vi "PicoScope5000aExampleStreamingMSO.vi"() -> ()   [LabVIEW 2016]
doc: "This example demonstrates how to use the PicoScope Labview library to stream data from a PicoScope 5000 Series Device"
uses:
  ps5000a.dll
  <vilib>/Waveform/DWDTOps.llb/DWDT Analog to Digital.vi
panel:
  out "Analog Channels":T1(graph)
  out "Raw Sample Interval (sec)":dbl=1.0000000130088963e-06 format="%#.5p"
  out "Max ADC value":i16
  out "Chunk time":u32
  out "Elapsed time":dbl
  in  "Poll time (ms)":u32=10 min=1 max=1000 step=1
  in  "Data file":path=path "PicoScope5000aExampleStreaming ChA Data"
  out "size(s)":i32
  out "Queue depth":i32(graph)
  out "queue depth":i32
  in  "Buffer and Transfer Settings":T2={"startIndex"=0, "Samples"=1000000, "Down Sample Ratio"=1, "Down-Sample Mode"=0} {"Down-Sample Mode" items=["None"=0, "Aggregate"=1, "Decimate"=2, "Average"=4]; "Down Sample Ratio" step=1; "Samples" format="%_6p"}
  in  "Channel A Settings":T3={"Enabled"=TRUE, "Coupling"=1, "Range"=6, "Analogue Offset"=0.0, "Bandwidth Limit"=0} {"Bandwidth Limit" items=["Full", "20MHz"]; "Range" items=["10 mV", "20 mV", "50 mV", "100 mV", "200 mV", "500 mV", "1 V", "2 V", "5 V", "10 V", "20 V"]; "Coupling" items=["AC", "DC"]}
  out "USB Powered":bool=TRUE
  out "USB 3.0 device on non-USB 3.0 Port":bool=TRUE
  out "TriggeredAt (In Buffer)":u32 format="%#.6p"
  out "TriggeredAt (Total samples)":u32 format="%#.6p"
  in  "Acquisition Settings":T4={"Auto Stop"=TRUE, "Desired Sample Interval"=1, "Pre-trigger Samples"=0, "Post-trigger Samples"=1000000, "Down-Sample Ratio"=1, "Down-Sample Mode"=0, "Time Units"=3} {"Time Units" items=["Nanoseconds (ns)"=2, "Microseconds (us)"=3, "Milliseconds (ms)"=4, "Seconds (s)"=5]; "Down-Sample Mode" items=["None"=0, "Aggregate"=1, "Decimate"=2, "Average"=4]; "Post-trigger Samples" format="%#.6p"; "Pre-trigger Samples" format="%#_6p"}
  out "Port 0":digitalwaveform(graph)={"t0"=timestamp(0 s since 1904-01-01), "dt"=1.0000000130088963e-06, "Y"={"transitions"=[], "data"=[]}}
  in  "Port 0 Settings":cluster{"Enabled":bool, "Logic Level":i16}={"Enabled"=FALSE, "Logic Level"=9830} {"Logic Level" items=["1.5V TTL"=9830, "2.5V CMOS"=16383]}
  in  "Trigger Settings":T5={"Trigger Enabled"=FALSE, "Trigger Source"=enum."Channel A", "Trigger Threshold (volts)"=0.0, "Trigger Direction"=2, "Trigger Delay (samples)"=0, "Auto Trigger Time (ms)"=1000} {"Trigger Direction" items=["Rising"=2, "Falling"=3]}
  out "Triggered":bool
  out "DownSample Interval (sec)":dbl=1.0000000130088963e-06 format="%#.5p"
  out "Total Samples":u32 format="%#.6p"
  out "Auto Stopped":bool
  in  "Serial Number":string
  in  "Open Using Serial Number":bool
  out "Number of Samples per Capture":u32 format="%#.6p"
  in  "Resolution":i32(ring) items=["8-bit", "12-bit", "14-bit", "15-bit (max. 2 ch.)", "16-bit (max. 1 ch.)"]
  in  "Apply  Settings":bool
  in  "stop":bool
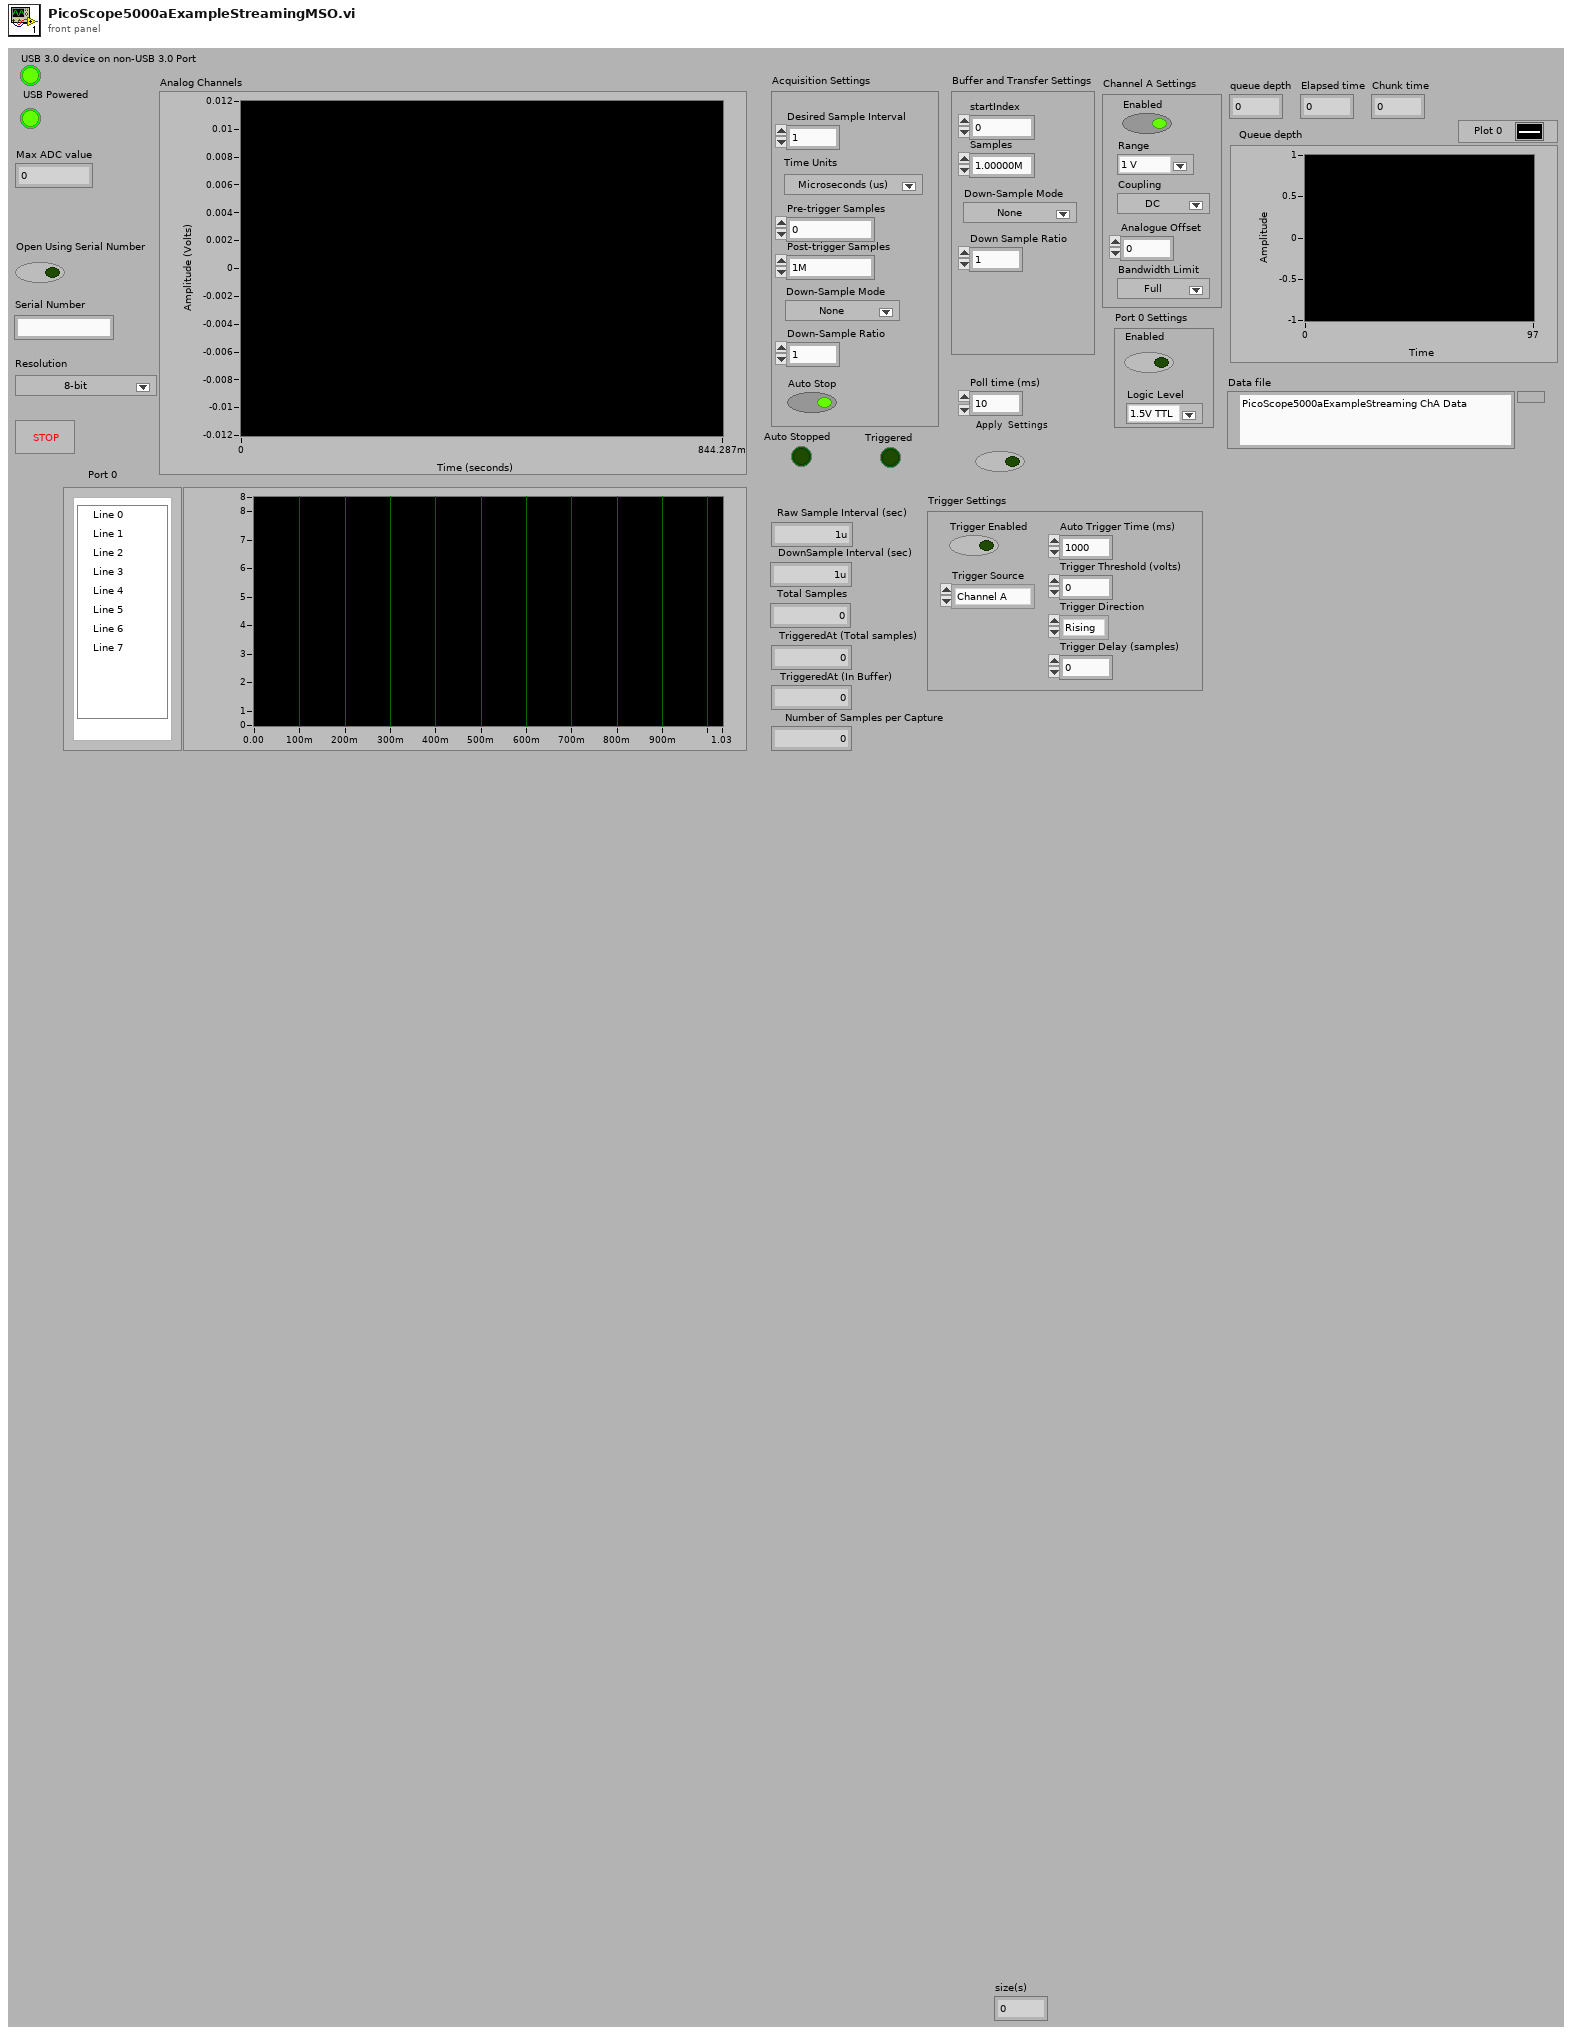
[diagram p1: front panel]
types:
  T1 = cluster{i32, "DownSample Interval (sec)":dbl, "Data":dbl[]}
  T2 = cluster{"startIndex":u64, "Samples":u64, "Down Sample Ratio":u64, "Down-Sample Mode":u32}
  T3 = cluster{"Enabled":bool, "Coupling":i16, "Range":u16, "Analogue Offset":sgl, "Bandwidth Limit":u32}
  T4 = cluster{"Auto Stop":bool, "Desired Sample Interval":u32, "Pre-trigger Samples":u32, "Post-trigger Samples":u32, "Down-Sample Ratio":u32, "Down-Sample Mode":i32, "Time Units":u32}
  T5 = cluster{"Trigger Enabled":bool, "Trigger Source":enum16{"Channel A", "Channel B", "Channel C", "Channel D", "Ext."}, "Trigger Threshold (volts)":dbl, "Trigger Direction":u16, "Trigger Delay (samples)":u32, "Auto Trigger Time (ms)":i16}
  T6 = enum16{"open", "open or create", "create or replace", "create", "open (read-only)"}
  T7 = cluster{"Driver Version":string, "USB Version":string, "Hardware":string, "Variant":string, "Batch and Serial":string, "Cal Date":string, "Kernel Version":string, "Digital HW Version":string, "Analogue HW Version":string, "MSO":bool, "Number of channels":i16}
  T8 = cluster{"Channel A Buffer":i16[], "Channel B Buffer":i16[], "Channel C Buffer":i16[], "Channel D Buffer":i16[], "Channel E Buffer":i16[], "Channel F Buffer":i16[], "Channel G Buffer":i16[], "Channel H Buffer":i16[], "Port 0":i16[], "Port 1":i16[]}
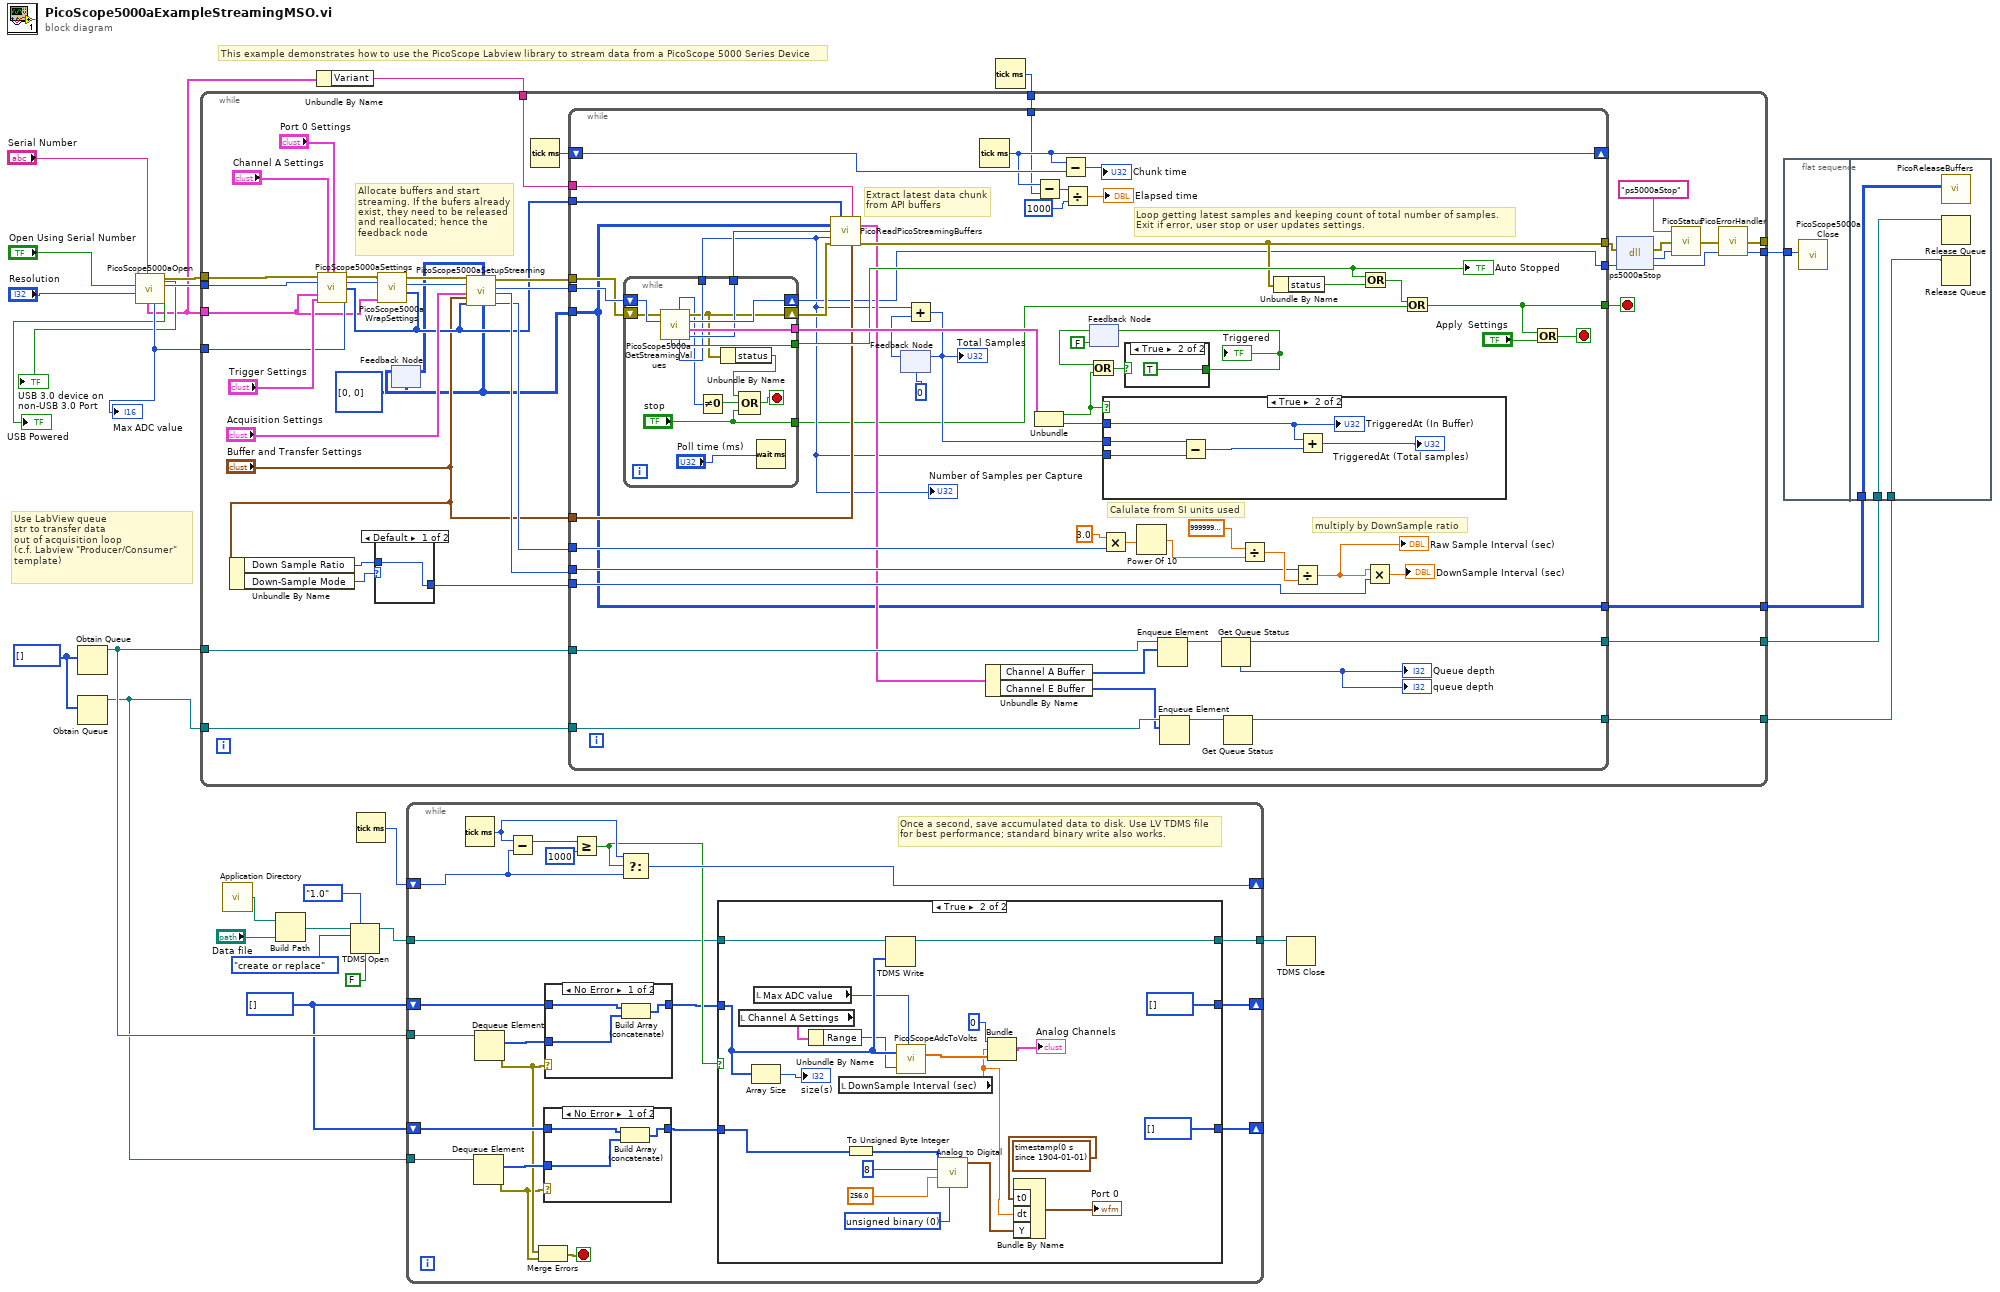
[diagram p0: block diagram]
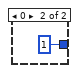
[diagram p5: hidden frame]
diagram:
  w6 = i16[] [] ("History Data")
  w9 = i16[] [] ("History Data")
  # "Use LabView queue\nstr to transfer data\nout of acquisition loop\n(c.f. Labview \"Producer/Consumer\"\ntemplate)"
  # "This example demonstrates how to use the PicoScope Labview library to stream data from a PicoScope 5000 Series Device"
  n1 = Obtain Queue(element data type=w9) -> (queue out=w22:refnum<queue>)  [unwired: 4 in, 2 out]
  n2 = Obtain Queue(element data type=w9) -> (queue out=w7:refnum<queue>)  [unwired: 4 in, 2 out]
  n3 = call "PicoScope5000aOpen.vi"("Serial Number"="Serial Number", "Resolution"="Resolution", "Use Serial Number"="Open Using Serial Number") -> ("USB Powered"=→"USB Powered":bool, "handle"=w27:i16, "error out"=w28:errorcluster, "Max ADC value"=w23:i16, "USB 3.0 device on non-USB 3.0 Port"=→"USB 3.0 device on non-USB 3.0 Port":bool, "Device Info"=w2:T7)  [unwired: 3 in]
  "Max ADC value" <- w23
  n4 = call <vilib>:"Application Directory.vi"() -> ("Application Directory"=w3:path)
  n5 = Build Path(base path=w3, name or relative path="Data file") -> (appended path=w4:path)
  n6 = Unbundle By Name(w2) -> ("Variant"=w1:string)
  n7 = TDMS Open(6:FALSE ("disable buffering? (T)"), 7:enum16{"1.0", "2.0"}."1.0" ("file format version (2.0)"), 10:T6."create or replace" ("operation (0:open)"), 11:w4) -> (3:w13:refnum<k34>)  [unwired: 3 in, 1 out]
  n8 = Tick Count (ms)() -> (millisecond timer value=w15:u32)
  n9 = while {
    tunnel: w22 -> [w48]
    shift-right: [w39] -> _
    shift-left: w6 -> [w47]
    shift-right: [w42] -> _
    shift-left: w15 -> [w43]
    tunnel: w13 -> [w38]
    tunnel: [w37] -> w12
    tunnel: w7 -> [w35]
    shift-right: [w32] -> _
    shift-left: w6 -> [w34]
    stop <- w31 stop-if-true
    # "Once a second, save accumulated data to disk. Use LV TDMS file\nfor best performance; standard binary write also works."
    n10 = Tick Count (ms)() -> (millisecond timer value=w44:u32)
    n11 = Dequeue Element(queue=w35) -> (element=w36:i16[], error out=w29:errorcluster)  [unwired: 2 in, 2 out]
    n12 = Dequeue Element(queue=w48) -> (element=w49:i16[], error out=w30:errorcluster)  [unwired: 2 in, 2 out]
    n13 = Subtract(x=w44, y=w43) -> (x-y=w46:u32)
    n14 = Merge Errors(w30, w29) -> (w31:errorcluster)
    n15 = case shown="No Error" w29 {
      tunnel: w34 -> [w52 w53]
      tunnel: [w51 w53] -> w33
      tunnel: w36 -> [w50 _]
      frame No Error {
        n16 = Build Array (concatenate)(w52, w50) -> (w51:i16[])
      }
      frame Error {
      }
    }
    n17 = case shown="No Error" w30 {
      tunnel: w47 -> [w80 w81]
      tunnel: [w79 w81] -> w40
      tunnel: w49 -> [w78 _]
      frame No Error {
        n18 = Build Array (concatenate)(w80, w78) -> (w79:i16[])
      }
      frame Error {
      }
    }
    n19 = Greater Or Equal?(x=w46, y=u32 1000) -> (x >= y?=w41:bool)
    n20 = Select(t=w44, s=w41, f=w43) -> (s? t:f=w42:u32)
    n21 = case shown="True" w41 {
      tunnel: w40 -> [w56 w73]
      tunnel: [w56 i16[] [] ("History Data")] -> w39
      tunnel: w38 -> [w55 w75]
      tunnel: [w55 w74] -> w37
      tunnel: w33 -> [w54 w59]
      tunnel: [w54 i16[] [] ("History Data")] -> w32
      frame False {
      }
      frame True {
        w65 = u16 0 items=["unsigned binary", "offset binary", "2's complement"] ("data format (offset binary)")
        n22 = local read "Channel A Settings"() -> (w69:T3)
        n23 = Array Size(array=w73) -> (size(s)=→"size(s)":i32)
        n24 = local read "Max ADC value"() -> (w68:i16)
        n25 = Unbundle By Name(w69) -> ("Range"=w72:u16)
        n26 = local read "DownSample Interval (sec)"() -> (w60:dbl)
        n27 = To Unsigned Byte Integer(number=w59) -> (unsigned 8bit integer=w64:u8[])
        n28 = TDMS Write(0:w75, 9:w73) -> (4:w74:refnum<k34>)  [unwired: 4 in, 3 out]
        n29 = call "PicoScopeAdcToVolts.vi"("Max_adc"=w68, "Range Index"=w72, "Data"=w73) -> ("Data"=w70:dbl[])
        n30 = call-poly <vilib>:"Analog to Digital.vi"("data format (offset binary)"=w65, "full-scale range (pk-pk)"=256.0, "resolution (16 bit)"=8, "analog waveform"=w64) -> ("digital waveform"=w61:digitalwaveform)  [unwired: 4 in, 3 out]
        n31 = Bundle(0, "DownSample Interval (sec)"=w60, "Data"=w70) -> (→"Analog Channels":T1)  [unwired: 1 in]
        n32 = Bundle By Name("t0"=timestamp(0 s since 1904-01-01), "dt"=w60, "Y"=w61) -> (→"Port 0":digitalwaveform)  [unwired: 1 in]
      }
    }
  }
  n33 = Tick Count (ms)() -> (millisecond timer value=w21:u32)
  n34 = while {
    tunnel: [w116] -> w20
    tunnel: w28 -> [w120]
    tunnel: w27 -> [w121]
    tunnel: w2 -> [w85]
    tunnel: w23 -> [w102]
    tunnel: [w94] -> w18
    tunnel: w22 -> [w93]
    tunnel: [w92] -> w19
    tunnel: [w90] -> _
    tunnel: w21 -> [w88]
    tunnel: [w84] -> w8
    tunnel: w7 -> [w83]
    tunnel: w1 -> [w82]
    stop <- w122 stop-if-true
    # "Allocate buffers and start\nstreaming. If the bufers already\nexist, they need to be released\nand reallocated; hence the\nfeedback node"
    n35 = Unbundle By Name("Buffer and Transfer Settings") -> ("Down Sample Ratio"=w99:u64, "Down-Sample Mode"=w101:u32)
    n36 = call "PicoScope5000aSettings.vi"("error in"=w120, "Channel A Settings"="Channel A Settings", "Port 0 Settings"="Port 0 Settings", "handle in"=w121, "Device Info"=w85, "Trigger Settings"="Trigger Settings", "Max ADC value"=w102) -> ("error out"=w109:errorcluster, "handle out"=w108:i16, "enabled array"=w96:i16[])  [unwired: 6 in]
    n37 = case shown="Default" w101 {
      tunnel: [w123 u32 1 ("Down-Sample Ratio")] -> w100
      tunnel: w99 -> [w123 _]
      frame Default {
      }
      frame 0 {
      }
    }
    n38 = call "PicoScope5000aWrapSettings.vi"("enabled array"=w96, "Device Info"=w85, "Handle In"=w108, "error in (no error)"=w109) -> ("Handle Out"=w111:i16, "error out"=w110:errorcluster)  [unwired: 6 in]
    n39 = feedback #1(u64[][] [[0], [0]] ("Pointer array")) -> (w91:u64[][])
    n40 = call "PicoScope5000aSetupStreaming.vi"("error in"=w110, "handle in"=w111, "Acquisition Settings"="Acquisition Settings", "Buffer and Transfer Settings"="Buffer and Transfer Settings", "enabled array"=w96, "Pointers In"=w91) -> ("Pointer array"=w87:u64[][], "error out"=w118:errorcluster, "handle out"=w119:i16, "Sample Interval"=w105:u32, "sampleIntervalTimeUnits"=w104:u32)  [unwired: 9 in]
    n41 = feedback-in #1(w87) -> ()
    n42 = Tick Count (ms)() -> (millisecond timer value=w89:u32)
    n43 = while {
      tunnel: [w135] -> w117
      tunnel: [w178] -> w122
      tunnel: w119 -> [w154]
      tunnel: w118 -> [w153]
      tunnel: w105 -> [w157]
      tunnel: w104 -> [w165]
      tunnel: [w150] -> w103
      tunnel: w100 -> [w155]
      tunnel: "Buffer and Transfer Settings" -> [w152]
      tunnel: w96 -> [w149]
      tunnel: [w147] -> w94
      tunnel: w93 -> [w145]
      tunnel: w87 -> [w143]
      tunnel: [w143] -> w92
      shift-right: [w138] -> _
      shift-left: w89 -> [w139]
      tunnel: w88 -> [w137]
      tunnel: w82 -> [w131]
      tunnel: [w128] -> w84
      tunnel: w83 -> [w127]
      stop <- w177 stop-if-true
      # "Loop getting latest samples and keeping count of total number of samples. \nExit if error, user stop or user updates settings."
      # "Extract latest data chunk\nfrom API buffers"
      # "Calulate from SI units used"
      # "multiply by DownSample ratio"
      n44 = while {
        tunnel: [w193] -> w176
        tunnel: [w192] -> w173
        tunnel: [w188] -> w133
        tunnel: [w187] -> w132
        shift-right: [w189] -> w135
        shift-left: w154 -> [w191]
        shift-right: [w186] -> w151
        shift-left: w153 -> [w190]
        tunnel: ["stop"] -> w125
        stop <- w181 stop-if-true
        n45 = call "PicoScope5000aGetStreamingValues.vi"("handle in"=w191, "error in"=w190) -> ("Start Index in Driver Buffer"=w188:u32, "Trigger"=w193:cluster{bool, "triggeredAt (Total samples)":u32}, "handle out"=w189:i16, "error out"=w186:errorcluster, "Number of Samples"=w187:u32, "ready"=w184:i16, "Auto Stopped"=w192:bool)  [unwired: 3 in]
        n46 = Not Equal To 0?(x=w184) -> (x != 0?=w182:bool)
        n47 = Unbundle By Name(w186) -> ("status"=w183:bool)
        n48 = Compound Arithmetic op=OR(w183, w182, "stop") -> (w181:bool)
        n49 = Wait (ms)(milliseconds to wait="Poll time (ms)") -> ()  [unwired: 1 out]
      }
      "Number of Samples per Capture" <- w132
      "Auto Stopped" <- w173
      n50 = call "PicoReadPicoStreamingBuffers.vi"("enabled array"=w149, "Buffer and Transfer Settings"=w152, "Variant"=w131, "Pointer array"=w143, "Offset Index"=w133, "Number of Samples"=w132, "error in (no error)"=w151) -> ("Buffers (Max or non-aggregated)"=w144:T8, "error out"=w150:errorcluster)  [unwired: 7 in]
      n51 = feedback #2(u32 0) -> (w169:u32)
      n52 = Add(x=w132, y=w169) -> (x+y=w161:u32)
      "Total Samples" <- w161
      n53 = feedback-in #2(w161) -> ()
      n54 = Tick Count (ms)() -> (millisecond timer value=w138:u32)
      n55 = Unbundle By Name(w144) -> ("Channel A Buffer"=w134:i16[], "Channel E Buffer"=w126:i16[])
      n56 = Subtract(x=w138, y=w137) -> (x-y=w142:u32)
      n57 = Unbundle(w176) -> (w159:bool, "triggeredAt (Total samples)"=w158:u32)
      n58 = Subtract(x=w138, y=w139) -> (x-y=→"Chunk time":u32)
      n59 = Divide(x=w142, y=u32 1000) -> (x/y=→"Elapsed time":dbl)
      n60 = feedback #3(FALSE) -> (w171:bool)
      n61 = Or(x=w171, y=w159) -> (x .or. y?=w162:bool)
      n62 = Multiply(x=3.0, y=w165) -> (x*y=w163:dbl)
      n63 = case shown="True" w159 {
        tunnel: w132 -> [_ w194]
        tunnel: w161 -> [_ w198]
        tunnel: w158 -> [_ w196]
        frame False {
        }
        frame True {
          n64 = Subtract(x=w198, y=w194) -> (x-y=w197:u32)
          n65 = Add(x=w196, y=w197) -> (x+y=→"TriggeredAt (Total samples)":u32)
          "TriggeredAt (In Buffer)" <- w196
        }
      }
      n66 = case shown="True" w162 {
        selector: w162 -> [w199 _]
        tunnel: [w199 TRUE] -> w160
        frame False {
        }
        frame True {
        }
      }
      "Triggered" <- w160
      n67 = feedback-in #3(w160) -> ()
      n68 = Power Of 10(x=w163) -> (10^x=w164:dbl)
      n69 = Enqueue Element(queue=w145, element=w134) -> (queue out=w146:refnum<queue>)  [unwired: 2 in, 2 out]
      n70 = Enqueue Element(queue=w127, element=w126) -> (queue out=w129:refnum<queue>)  [unwired: 2 in, 2 out]
      n71 = Get Queue Status(queue=w146) -> (queue out=w147:refnum<queue>, # elements in queue=→"queue depth" →"Queue depth":i32)  [unwired: 2 in, 6 out]
      n72 = Get Queue Status(queue=w129) -> (queue out=w128:refnum<queue>)  [unwired: 2 in, 7 out]
      n73 = Divide(x=sgl 1000000000000000.0 ("y"), y=w164) -> (x/y=w166:dbl)
      n74 = Unbundle By Name(w150) -> ("status"=w175:bool)
      n75 = Divide(x=w157, y=w166) -> (x/y=w130:dbl)
      "Raw Sample Interval (sec)" <- w130
      n76 = Or(x=w173, y=w175) -> (x .or. y?=w174:bool)
      n77 = Multiply(x=w130, y=w155) -> (x*y=→"DownSample Interval (sec)":dbl)
      n78 = Or(x=w174, y=w125) -> (x .or. y?=w178:bool)
      n79 = Or(x=w178, y="Apply  Settings") -> (x .or. y?=w177:bool)
    }
    n80 = dll-call lib="ps5000a.dll" fn="ps5000aStop"(error in=w103, "handle"=w117) -> (error out=w114:errorcluster, "PICO_STATUS"=w115:u32, "handle"=w116:i16)  [unwired: 2 in, 1 out]
    n81 = call "PicoStatus.vi"("PICO STATUS"=w115, "error in"=w114, "source"="ps5000aStop") -> ("error out"=w113:errorcluster)
    n82 = call "PicoErrorHandler.vi"("error in"=w113) -> ("error out"=w90:errorcluster)
  }
  n83 = TDMS Close(11:w12) -> ()  [unwired: 1 in, 2 out]
  n84 = flat-sequence {
    tunnel: w20 -> [w201]
    tunnel: w19 -> [w204]
    tunnel: w18 -> [w203]
    tunnel: w8 -> [w202]
    frame #0 {
      n85 = call "PicoScope5000aClose.vi"("handle"=w201) -> ()
    }
    frame #1 {
      n86 = call "PicoReleaseBuffers.vi"("Pointer array"=w204) -> ()  [unwired: 10 in, 1 out]
      n87 = Release Queue(queue=w203) -> ()  [unwired: 2 in, 3 out]
      n88 = Release Queue(queue=w202) -> ()  [unwired: 2 in, 3 out]
    }
  }
